vi "add to point buffer.vi"(9 "value":dbl, 10 "time":timestamp, 11 "point buffer":refnum<data-value>) -> (0 "error out":errorcluster)   [LabVIEW 2020, in "nominal core steps.lvlib"]
doc: "Add a single time/value point to the buffer."
uses:
  nominal core steps.lvlib
  points buffer.ctl
  single point.ctl
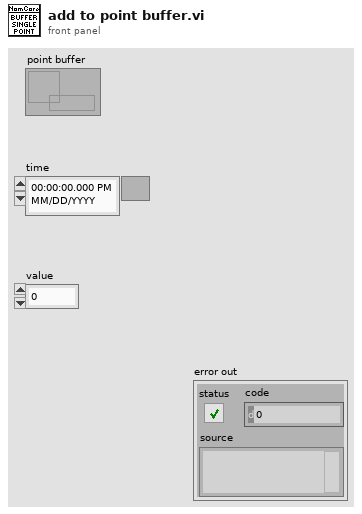
[diagram p1: front panel]
types:
  T1 = typedef "nominal core steps.lvlib/single point.ctl" = cluster{"Time Stamp":timestamp, "Value":dbl}
  T2 = typedef "nominal core steps.lvlib/points buffer.ctl" = T1[]
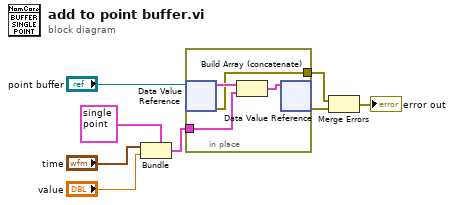
[diagram p0: block diagram]
diagram:
  n1 = Bundle(cluster=T1 {"Time Stamp"=timestamp(0 s since 1904-01-01), "Value"=0.0} ("Point"), "Time Stamp"="time", "Value"="value") -> (w5:T1)
  n2 = in-place {
    in-place-border: w5 -> [w10]
    in-place-border: [w9] -> w3
    n3 = in-place-dvr #1("point buffer") -> (w12:T2, w9:errorcluster)
    n4 = Build Array (concatenate)(w12, w10) -> (w11:T2)
    n5 = in-place-dvr #1(w11) -> (w4:errorcluster)  [unwired: 1 out]
  }
  n6 = Merge Errors(w3, w4) -> (→"error out":errorcluster)
